vi "Update Displays.vi"(8 "error in":errorcluster, 10 "Status":string, 11 "Sequence Executor in":refnum<class "Sequence Executor.lvclass">) -> (0 "error out":errorcluster, 3 "Sequence Executor out":refnum<class "Sequence Executor.lvclass">)   [LabVIEW 2026, in "Sequence Executor.lvclass"]
doc: "PRIVATE. Writes the given Status, Current Step (Step Index + 1), Step Table (Build Step Table of Sequence + Results) and Overall Verdict through the stored display refs. Display-write errors are swallowed (invalid refs tolerated). Does not change the object data."
uses:
  Sequence Executor.lvclass
  Sequence Executor.lvclass/Sequence Executor.ctl
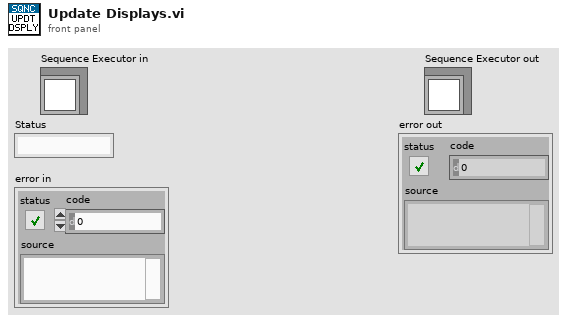
[diagram p1: front panel]
types:
  T1 = typedef "Sequence File.ctl" = cluster{"sequence_id":string, "description":string, "rig_config":string, "steps":T2[]}
  T2 = typedef "Step Config.ctl" = cluster{"step_no":i32, "step_name":string, "command_type":string, "setpoints":T3[], "conditions":T4[], "dwell_time_ms":i32, "timeout_ms":i32, "expected_result":string}
  T3 = typedef "Channel Value.ctl" = cluster{"channel":string, "value":dbl}
  T4 = typedef "Condition.ctl" = cluster{"channel":string, "target":dbl, "tolerance":dbl}
  T5 = typedef "Step Result.ctl" = cluster{"step_no":i32, "step_name":string, "result":string, "reason":string, "measured":dbl, "target":dbl, "duration_ms":dbl}
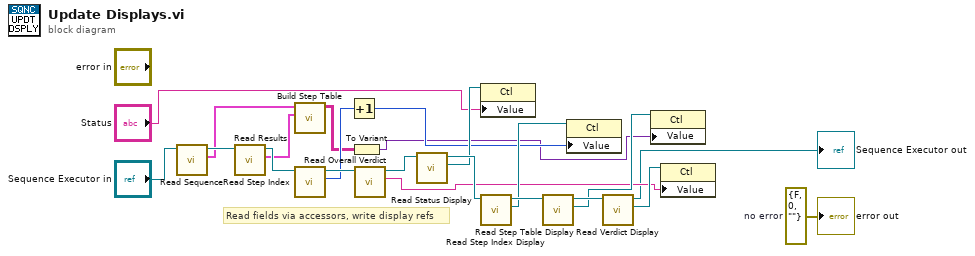
[diagram p0: block diagram]
diagram:
  w1 = errorcluster {"status"=FALSE, "code"=0, "source"=""}  # no error
  # "Read fields via accessors, write display refs"
  n1 = call "Read Sequence.vi"("Sequence Executor in"="Sequence Executor in") -> ("Sequence File"=w14:T1, "Sequence Executor out"=w21:refnum<class "Sequence Executor.lvclass">)  [unwired: 8 in, 1 out]
  n2 = call "Read Results.vi"("Sequence Executor in"=w21) -> ("Results"=w13:T5[], "Sequence Executor out"=w20:refnum<class "Sequence Executor.lvclass">)  [unwired: 8 in, 1 out]
  n3 = call "Build Step Table.vi"("Step Results"=w13, "Sequence File"=w14) -> ("Step Table"=w7:string[][])  [unwired: 9 in]
  n4 = call "Read Step Index.vi"("Sequence Executor in"=w20) -> ("Step Index"=w12:i32, "Sequence Executor out"=w19:refnum<class "Sequence Executor.lvclass">)  [unwired: 8 in, 1 out]
  n5 = Increment(x=w12) -> (x+1=w8:i32)
  n6 = To Variant(anything=w7) -> (Variant=w5:variant)
  n7 = call "Read Overall Verdict.vi"("Sequence Executor in"=w19) -> ("Overall Verdict"=w3:string, "Sequence Executor out"=w18:refnum<class "Sequence Executor.lvclass">)  [unwired: 8 in, 1 out]
  n8 = call "Read Status Display.vi"("Sequence Executor in"=w18) -> ("Status Display"=w11:refnum<vi>, "Sequence Executor out"=w17:refnum<class "Sequence Executor.lvclass">)  [unwired: 8 in, 1 out]
  n9 = property class="Ctl"(reference=w11, "Value"="Status") -> ()  [unwired: 1 in, 2 out]
  n10 = call "Read Step Index Display.vi"("Sequence Executor in"=w17) -> ("Step Index Display"=w9:refnum<vi>, "Sequence Executor out"=w16:refnum<class "Sequence Executor.lvclass">)  [unwired: 8 in, 1 out]
  n11 = call "Read Step Table Display.vi"("Sequence Executor in"=w16) -> ("Step Table Display"=w6:refnum<vi>, "Sequence Executor out"=w15:refnum<class "Sequence Executor.lvclass">)  [unwired: 8 in, 1 out]
  n12 = property class="Ctl"(reference=w9, "Value"=w8) -> ()  [unwired: 1 in, 2 out]
  n13 = call "Read Verdict Display.vi"("Sequence Executor in"=w15) -> ("Verdict Display"=w4:refnum<vi>, "Sequence Executor out"=→"Sequence Executor out":refnum<class "Sequence Executor.lvclass">)  [unwired: 8 in, 1 out]
  n14 = property class="Ctl"(reference=w6, "Value"=w5) -> ()  [unwired: 1 in, 2 out]
  n15 = property class="Ctl"(reference=w4, "Value"=w3) -> ()  [unwired: 1 in, 2 out]
  "error out" <- w1
